vi "Day 16-Parse Input.vi"(11 "String in":string) -> (3 "String out":string)   [LabVIEW 2021]
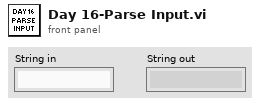
[diagram p1: front panel]
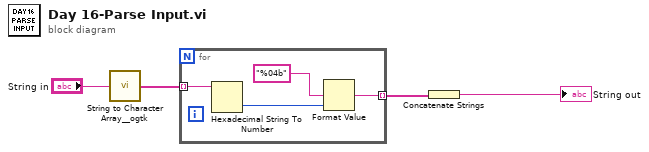
[diagram p0: block diagram]
diagram:
  n1 = call <userlib>:"String to Character Array__ogtk.vi"("Input String"="String in") -> ("Character Array"=w2:string[])
  n2 = for {
    tunnel: w2 -> [w8] mode=indexing
    tunnel: [w5] -> w3 mode=indexing
    n3 = Hexadecimal String To Number(string=w8) -> (number=w6:u32)  [unwired: 2 in, 1 out]
    n4 = Format Value(format string="%04b", value (0)=w6) -> (output string=w5:string)  [unwired: 1 in]
  }
  n5 = Concatenate Strings(w3) -> (→"String out":string)
